vi "Route 3D Controller Command.vi"(8 "error in (no error)":errorcluster caption="에러 입력(에러 없음)", 10 "문자열":string, 11 "Instrument Manager 입력":refnum<class "Instrument Manager.lvclass">) -> (0 "error out":errorcluster caption="에러 출력", 3 "Instrument Manager 출력":refnum<class "Instrument Manager.lvclass">)   [LabVIEW 2023, in "Instrument Manager.lvclass"]
uses:
  Instrument Manager.lvclass
  <vilib>/regexp/Match Regular Expression.xnode
  Instrument Manager.lvclass/Instrument Manager.ctl
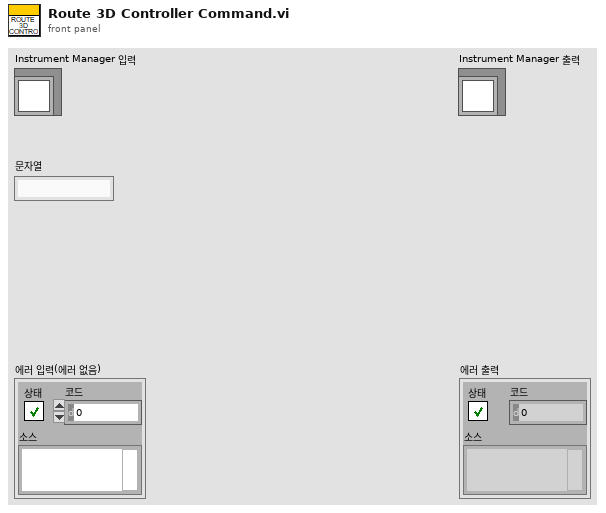
[diagram p1: front panel]
types:
  T1 = typedef "Instrument Manager.lvclass/Connect 3D Controller Param.ctl" = cluster{"type":string, "id":string, "target":string, "command":string, "Params":cluster{"VISA Resource":string}}
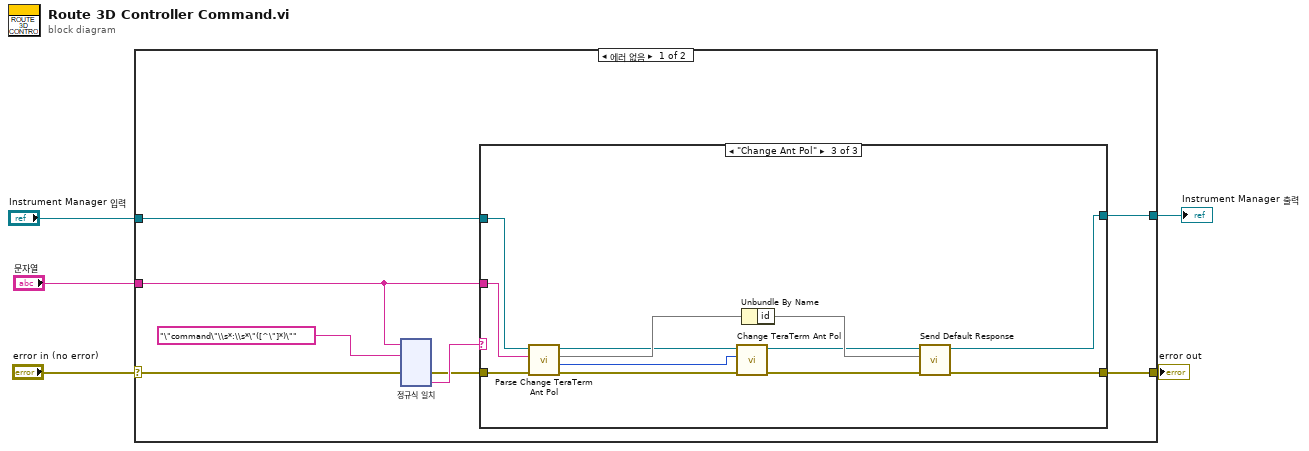
[diagram p0: block diagram]
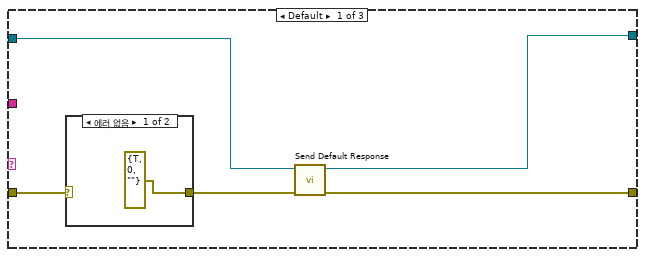
[diagram p2: hidden frame]
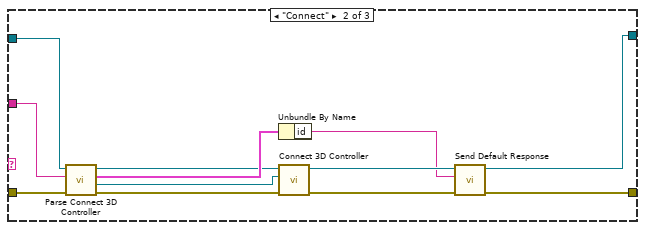
[diagram p4: hidden frame]
diagram:
  n1 = case shown="에러 없음" "error in (no error)" {
    selector: "error in (no error)" -> [w12 w165]
    tunnel: [w8 w165] -> w4
    tunnel: [w6 w164] -> w2
    tunnel: "Instrument Manager 입력" -> [w7 w164]
    tunnel: "문자열" -> [w9 _]
    frame No Error {
      n2 = xnode "정규식 일치"("입력 문자열"=w9, "정규식"="\"command\"\\s*:\\s*\"([^\"]*)\"", "에러 입력"=w12) -> ("에러 출력"=w10:errorcluster, "부분 일치 1"=w11:string)  [unwired: 3 in, 4 out]
      n3 = case shown="\"Change Ant Pol\"" w11 {
        tunnel: w10 -> [w17 w32 w42]
        tunnel: w9 -> [_ w30 w43]
        tunnel: [w16 w23 w40] -> w8
        tunnel: w7 -> [w15 w29 w44]
        tunnel: [w14 w22 w38] -> w6
        frame Default {
          n4 = case shown="에러 없음" w17 {
            selector: w17 -> [_ w20]
            tunnel: [errorcluster {"status"=TRUE, "code"=0, "source"=""} ("error IO") w20] -> w18
            frame No Error {
            }
            frame Error {
            }
          }
          n5 = call "Send Default Response.vi"("error in (no error)"=w18, "Instrument Manager 입력"=w15) -> ("error out"=w16:errorcluster, "Instrument Manager 출력"=w14:refnum<class "Instrument Manager.lvclass">)  [unwired: 8 in]
        }
        frame "Connect" {
          n6 = call "Parse Connect 3D Controller.vi"("error in (no error)"=w32, "JSON string"=w30, "Instrument Manager 입력"=w29) -> ("error out"=w26:errorcluster, "VISA 리소스 이름"=w27:refnum<visa-resource-name>, "Connect 3D Controller Param"=w31:T1, "Instrument Manager 출력"=w28:refnum<class "Instrument Manager.lvclass">)  [unwired: 5 in]
          n7 = Unbundle By Name(w31) -> ("id"=w21:string)
          n8 = call "Connect 3D Controller.vi"("error in (no error)"=w26, "VISA resource name"=w27, "Instrument Manager 입력"=w28) -> ("error out"=w25:errorcluster, "Instrument Manager 출력"=w24:refnum<class "Instrument Manager.lvclass">)  [unwired: 6 in, 1 out]
          n9 = call "Send Default Response.vi"("error in (no error)"=w25, "id"=w21, "Instrument Manager 입력"=w24) -> ("error out"=w23:errorcluster, "Instrument Manager 출력"=w22:refnum<class "Instrument Manager.lvclass">)  [unwired: 7 in]
        }
        frame "Change Ant Pol" {
          n10 = call "Parse Change TeraTerm Ant Pol.vi"("error in (no error)"=w42, "JSON string"=w43, "Instrument Manager 입력"=w44) -> ("error out"=w33:errorcluster, "Antenna Pol"=w34:enum16{"H", "V"}, 2:w41, "Instrument Manager 출력"=w35:refnum<class "Instrument Manager.lvclass">)  [unwired: 5 in]
          n11 = call "Change TeraTerm Ant Pol.vi"("error in (no error)"=w33, "Antenna Pol"=w34, "Instrument Manager 입력"=w35) -> ("error out"=w37:errorcluster, "Instrument Manager 출력"=w36:refnum<class "Instrument Manager.lvclass">)  [unwired: 7 in]
          n12 = Unbundle By Name(w41) -> ("id"=w39)
          n13 = call "Send Default Response.vi"("error in (no error)"=w37, "id"=w39, "Instrument Manager 입력"=w36) -> ("error out"=w40:errorcluster, "Instrument Manager 출력"=w38:refnum<class "Instrument Manager.lvclass">)  [unwired: 7 in]
        }
      }
    }
    frame Error {
    }
  }
  "error out" <- w4
  "Instrument Manager 출력" <- w2
